vi "Test MQTT-3.8.1-1.vi"(8 "error in (no error)":errorcluster, 11 "Connection Config":refnum<class "Connection.lvclass">) -> (0 "error out":errorcluster, 3 "Connection Config dup":refnum<class "Connection.lvclass">)   [LabVIEW 2013]
uses:
  <vilib>/LabVIEW Open Source Project/MQTT Connection/MQTT_Connection/Connection/Connection.lvclass
  <vilib>/LabVIEW Open Source Project/MQTT Control Packets/Control Packets/SUBSCRIBE/Topic Subscription -- cluster.ctl
  <vilib>/LabVIEW Open Source Project/MQTT Control Packets/Control Packets/ControlPacket/QualityOfService -- enum.ctl
  <vilib>/LabVIEW Open Source Project/MQTT Control Packets/Control Packets/ControlPacket/ControlPacket.lvclass/ControlPacket.ctl
  <vilib>/addons/_JKI Toolkits/Caraya/classes/Test/Test.lvclass
  <vilib>/LabVIEW Open Source Project/MQTT Client/Client class/Client.lvclass
  <vilib>/LabVIEW Open Source Project/MQTT Control Packets/Control Packets/SUBSCRIBE/SUBSCRIBE.lvclass
  <vilib>/LabVIEW Open Source Project/MQTT Control Packets/Control Packets/ControlPacket/ControlPacket.lvclass
  <vilib>/addons/_JKI Toolkits/Caraya/classes/Assert/Assert.lvclass
  <vilib>/LabVIEW Open Source Project/MQTT Connection/MQTT_Base/Base Class/MQTT_Base.lvclass
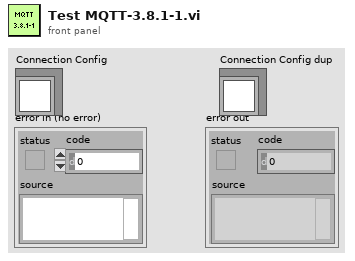
[diagram p1: front panel]
types:
  T1 = typedef "MQTT_Control_Packets.lvlib/SUBSCRIBE.lvclass/Topic Subscription -- cluster.ctl" = cluster{"Topic Filter":string, "QoS":T2}
  T2 = typedef "MQTT_Control_Packets.lvlib/ControlPacket.lvclass/QualityOfService -- enum.ctl" = enum16{"0 (At Most Once)", "1 (At Least Once)", "2 (Exactly Once)"}
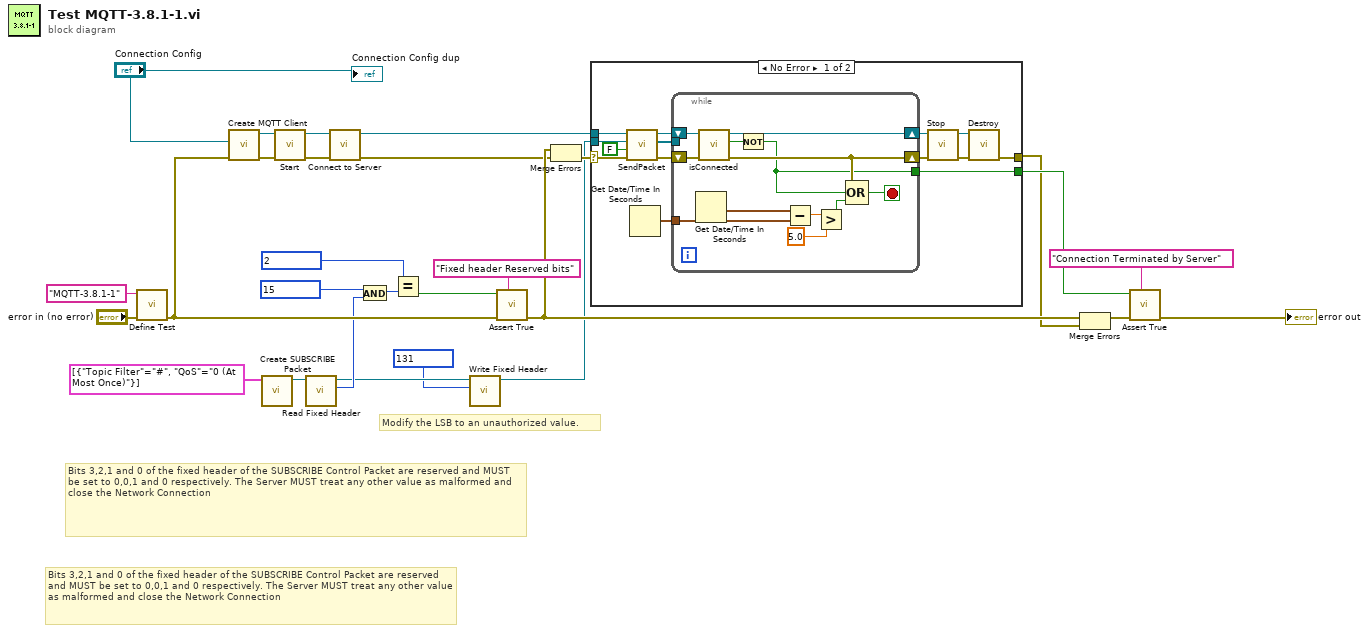
[diagram p0: block diagram]
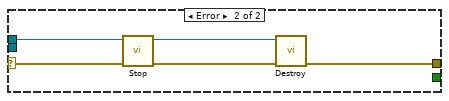
[diagram p2: hidden frame]
diagram:
  # "Modify the LSB to an unauthorized value."
  # "Bits 3,2,1 and 0 of the fixed header of the SUBSCRIBE Control Packet are reserved and MUST be set to 0,0,1 and 0 respectively. The Server MUST treat any other value as malformed and close the Network Connection"
  # "Bits 3,2,1 and 0 of the fixed header of the SUBSCRIBE Control Packet are reserved and MUST be set to 0,0,1 and 0 respectively. The Server MUST treat any other value as malformed and close the Network Connection"
  n1 = call <vilib>:"Define Test.vi"("error in (no error)"="error in (no error)", "Label (VI Title)"="MQTT-3.8.1-1") -> ("error out"=w20:errorcluster)  [unwired: 9 in]
  n2 = call <vilib>:"Create MQTT Client.vi"("error in (no error)"=w20, "Connection Configuration"="Connection Config") -> ("error out"=w4:errorcluster, "Client out"=w6:refnum<class "Client.lvclass">)  [unwired: 8 in]
  n3 = call <vilib>:"Create SUBSCRIBE Packet.vi"("Topic Subscriptions"=T1[] [{"Topic Filter"="#", "QoS"=enum."0 (At Most Once)"}]) -> ("SUBSCRIBE out"=w23:refnum<class "SUBSCRIBE.lvclass">)  [unwired: 8 in, 2 out]
  n4 = call <vilib>:"Start.vi"("error in (no error)"=w4, "MQTT_Base in"=w6) -> ("error out"=w3:errorcluster, "MQTT_Base out"=w5:refnum<class "Client.lvclass">)  [unwired: 7 in, 1 out]
  n5 = call <vilib>:"Read Fixed Header.vi"("ControlPacket in"=w23) -> ("Fixed Header"=w16:u8, "ControlPacket out"=w11:refnum<class "SUBSCRIBE.lvclass">)  [unwired: 9 in]
  n6 = call <vilib>:"Connect to Server.vi"("error in (no error)"=w3, "Client in"=w5) -> ("error out"=w8:errorcluster, "Client out"=w7:refnum<class "Client.lvclass">)  [unwired: 6 in, 2 out]
  n7 = And(x=u8 15, y=w16) -> (x .and. y?=w14:u8)
  n8 = Equal?(x=u8 2, y=w14) -> (x = y?=w12:bool)
  n9 = call <vilib>:"Write Fixed Header.vi"("Fixed Header"=u8 131, "ControlPacket in"=w11) -> ("ControlPacket out"=w10:refnum<class "SUBSCRIBE.lvclass">)  [unwired: 9 in]
  n10 = call <vilib>:"Assert True.vi"("Label"="Fixed header Reserved bits", "error in (no error)"=w20, "True?"=w12) -> ("error out"=w18:errorcluster)  [unwired: 8 in]
  n11 = Merge Errors(w18, w8) -> (w17:errorcluster)
  n12 = case shown="No Error" w17 {
    selector: w17 -> [w40 w56]
    tunnel: w7 -> [w41 w58]
    tunnel: [w42 w59] -> w1
    tunnel: [w32 _] -> w24
    tunnel: w10 -> [w39 _]
    frame No Error {
      n13 = call <vilib>:"SendPacket.vi"("error in (no error)"=w40, "Wait for ack? (T)"=FALSE, "ControlPacket"=w39, "Client in"=w41) -> ("error out"=w35:errorcluster, "Response"=w30:refnum<class "ControlPacket.lvclass">[], "Client out"=w36:refnum<class "Client.lvclass">)  [unwired: 5 in]
      n14 = Get Date/Time In Seconds() -> (seconds since 1Jan1904=w31:timestamp)
      n15 = while {
        shift-right: [w51] -> w34
        shift-left: w35 -> [w52]
        shift-right: [w53] -> w33
        shift-left: w36 -> [w54]
        tunnel: [w48] -> w32
        tunnel: w31 -> [w43]
        tunnel: w30 -> [_]
        stop <- w50 stop-if-true
        n16 = Get Date/Time In Seconds() -> (seconds since 1Jan1904=w44:timestamp)
        n17 = call <vilib>:"isConnected.vi"("error in (no error)"=w52, "Client in"=w54) -> ("error out"=w51:errorcluster, "connected"=w49:bool, "Client out"=w53:refnum<class "Client.lvclass">)  [unwired: 7 in]
        n18 = Not(x=w49) -> (.not. x?=w48:bool)
        n19 = Subtract(x=w44, y=w43) -> (x-y=w47:dbl)
        n20 = Greater?(x=w47, y=5.0) -> (0:w45:bool)
        n21 = Compound Arithmetic op=OR(w51, w48, w45) -> (w50:bool)
      }
      n22 = call <vilib>:"Stop.vi"("error in (no error)"=w34, "MQTT_Base in"=w33) -> ("error out"=w37:errorcluster, "MQTT_Base out"=w38:refnum<class "Client.lvclass">)  [unwired: 7 in, 1 out]
      n23 = call <vilib>:"Destroy.vi"("error in (no error)"=w37, "MQTT_Base in"=w38) -> ("error out"=w42:errorcluster)  [unwired: 8 in, 1 out]
    }
    frame Error {
      n24 = call <vilib>:"Stop.vi"("error in (no error)"=w56, "MQTT_Base in"=w58) -> ("error out"=w55:errorcluster, "MQTT_Base out"=w57:refnum<class "Client.lvclass">)  [unwired: 7 in, 1 out]
      n25 = call <vilib>:"Destroy.vi"("error in (no error)"=w55, "MQTT_Base in"=w57) -> ("error out"=w59:errorcluster)  [unwired: 8 in, 1 out]
    }
  }
  n26 = Merge Errors(w18, w1) -> (w19:errorcluster)
  n27 = call <vilib>:"Assert True.vi"("Label"="Connection Terminated by Server", "error in (no error)"=w19, "True?"=w24) -> ("error out"=→"error out":errorcluster)  [unwired: 8 in]
  "Connection Config dup" <- "Connection Config"
